vi "[ce] Integration.vi"(6 "parameters":cluster{"name":string, "value":dbl}[](array[cluster]) {"value" format="%.2f"}, 7 "# points":u32=200, 8 "error in":errorcluster, 9 "formula info":cluster{"formula":string, "x-variable":string}={"formula"="", "x-variable"="x"}, 10 "end":dbl=1.0 format="%.2f", 11 "start":dbl format="%.2f") -> (0 "error out":errorcluster, 1 "Integral of Y":dbl[](array[numeric]) format="%.2f", 2 "Y Values":dbl[](array[numeric]) format="%.2f", 3 "X Values":dbl[](array[numeric]) format="%.2f", 4 "ticks":u32)   [LabVIEW 2021]
doc: "Calculates both function values and the values of the integral of 1D function defined by a formula. In addition, the VI allows specifying additional parameters and evaluating them in formula.\nThe VI uses an algorithm based on solving of ordinary differential equations with the help of the Runge Kutta method.\n\n::: CalcExpress Toolkit :::\nCopyright (c) 2000-2026 Konstantin Shifershteyn. All rights reserved."
panel:
  # "Example 1:\n---------------\nformula info:\n  formula: sin(t*t)+t\n  x-variable: t\nparameters:  empty array\n\nExample 2:\n---------------\nformula info:\n  formula: a*sin(x)*exp(-x/b)\n  x-variable: x\nparameters: (a,1), (b,2)"
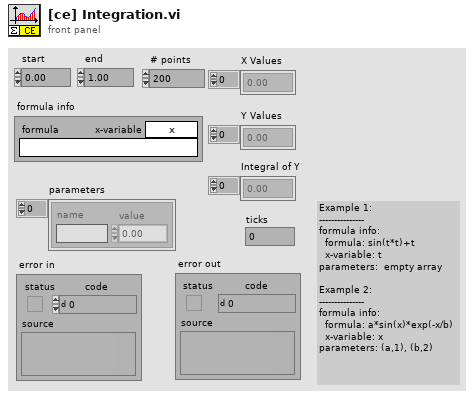
[diagram p1: front panel]
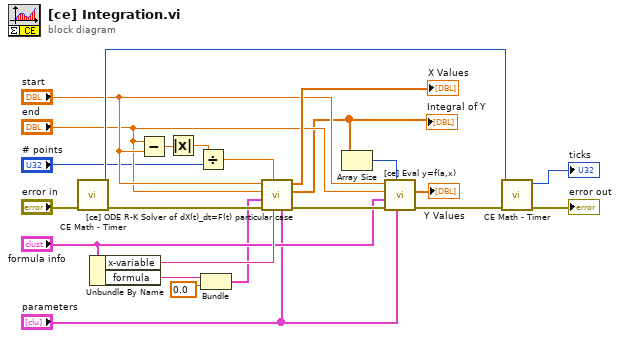
[diagram p0: block diagram]
diagram:
  n1 = call "CE Math - Timer.vi"("error in (no error)"="error in") -> ("error out"=w14:errorcluster, "ticks out"=w10:u32)  [unwired: 7 in]
  n2 = Unbundle By Name("formula info") -> ("x-variable"=w20:string, "formula"=w4:string)
  n3 = Subtract(x="end", y="start") -> (x-y=w22:dbl)
  n4 = Absolute Value(x=w22) -> (abs(x)=w23:dbl)
  n5 = Divide(x=w23, y="# points") -> (x/y=w6:dbl)
  n6 = Bundle("formula"=w4, "init value"=0.0) -> (w2:cluster{"formula":string, "init value":dbl})  [unwired: 1 in]
  n7 = call "[ce] ODE R-K Solver of dX(t)_dt=F(t) particular case.vi"("parameters"="parameters", "time"=w20, "h (step rate)"=w6, "error in"=w14, "equation info"=w2, "time end"="end", "time start"="start") -> ("error out"=w19:errorcluster, "X Values (solution)"=w1:dbl[], "Times"=→"X Values":dbl[])  [unwired: 1 in, 1 out]
  "Integral of Y" <- w1
  n8 = Array Size(array=w1) -> (size(s)=w18:i32)
  n9 = call "[ce] Eval y=f(a,x).vi"("parameters"="parameters", "# points"=w18, "error in"=w19, "formula info"="formula info", "end"="end", "start"="start") -> ("error out"=w13:errorcluster, "Y Values"=→"Y Values":dbl[])  [unwired: 2 in, 2 out]
  n10 = call "CE Math - Timer.vi"("error in (no error)"=w13, "ticks in"=w10) -> ("error out"=→"error out":errorcluster, "ticks out"=→"ticks":u32)  [unwired: 6 in]
